vi "variant to double.vi"(1 "Variant":variant) -> (0 "Double":dbl)   [LabVIEW 2025]
doc: "convert variant data to a LabVIEW Double\n<B>Input:</B>\nVariant (skalar)\n<B>Output:</B>\nDouble"
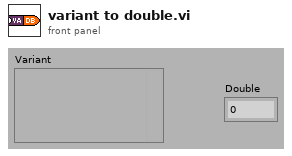
[diagram p1: front panel]
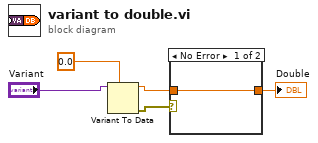
[diagram p0: block diagram]
diagram:
  n1 = Variant To Data(type=0.0 ("MIN U/36V"), Variant="Variant") -> (data=w4:dbl, error out=w3:errorcluster)  [unwired: 1 in]
  n2 = case shown="No Error" w3 {
    tunnel: w4 -> [w6 _]
    tunnel: [w6 _] -> w5
    frame No Error {
    }
    frame Error {
    }
  }
  "Double" <- w5
